vi "TCP_Acquisition.vi"() -> ()   [LabVIEW 2026]
panel:
  out "tcp_connected":bool
  in  "stop_acquisition":bool
  out "tcp_recieved_data":string
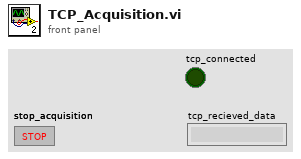
[diagram p1: front panel]
types:
  T1 = enum16{"Standard", "Buffered", "CRLF", "Immediate"}
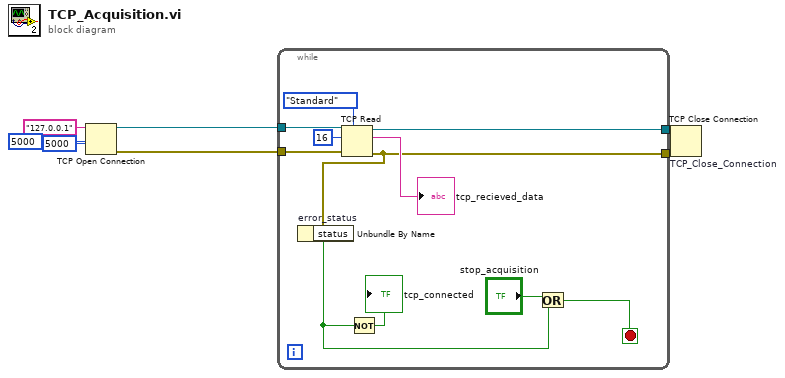
[diagram p0: block diagram]
diagram:
  n1 = TCP Open Connection(address="127.0.0.1", remote port or service name=u16 5000, timeout ms (60000)=5000) -> (connection ID=w4:refnum<k5>, error out=w3:errorcluster)  [unwired: 2 in]
  n2 = while {
    tunnel: w4 -> [w18]
    tunnel: w3 -> [w17]
    tunnel: [w15] -> w2
    tunnel: [w12] -> w1
    stop <- w10 stop-if-true
    n3 = TCP Read(connection ID=w18, bytes to read=16, error in (no error)=w17, 7:T1."Standard" ("mode (standard)")) -> (connection ID out=w15:refnum<k5>, data out=→"tcp_recieved_data":string, error out=w12:errorcluster)  [unwired: 1 in]
    n4 = Unbundle By Name "error_status"(w12) -> ("status"=w9:bool)
    n5 = Not(x=w9) -> (.not. x?=→"tcp_connected":bool)
    n6 = Or(x="stop_acquisition", y=w9) -> (x .or. y?=w10:bool)
  }
  n7 = TCP Close Connection "TCP_Close_Connection"(connection ID=w2, error in (no error)=w1) -> ()  [unwired: 1 in, 2 out]
